vi "Startup.vi"(6 "LabVIEW Web Service":refnum<class "Web Service.lvclass">) -> ()   [LabVIEW 2015]
uses:
  <vilib>/wsapi/Web Service.lvclass
  Configuration/Global_Configurations.vi
panel:
  # "Use the web service input terminal to call the VIs on the Service subpalette of the Web Services palette. Do not remove it from the connector pane unless you don't need access to the palette."
  # "Any additional terminals added to the connector pane of a startup VI will be ignored."
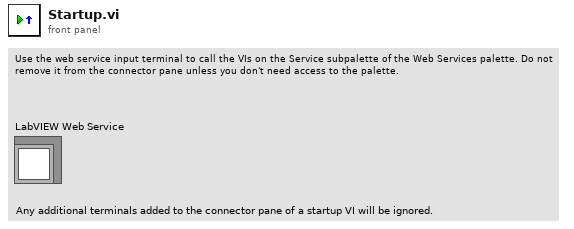
[diagram p1: front panel]
types:
  T1 = cluster{"Path":path, "Name":string, "Authors":string, "Keywords":string, "Description":string, "Cameras":cluster{"Base URL":string, "Path":string, "Name":string}[], "Sampling":cluster{"Sampled Variable":string, "Delta":dbl, "Sampling Freq":u32}[]}[]
  T2 = cluster{"Path":path, "Name":string, "Authors":string, "Keywords":string, "Description":string, "Cameras":cluster{"Base URL":string, "Path":string, "Name":string}[], "Sampling":cluster{"Sampled Variable":string, "Delta":dbl, "Sampling Freq":u32}[]}
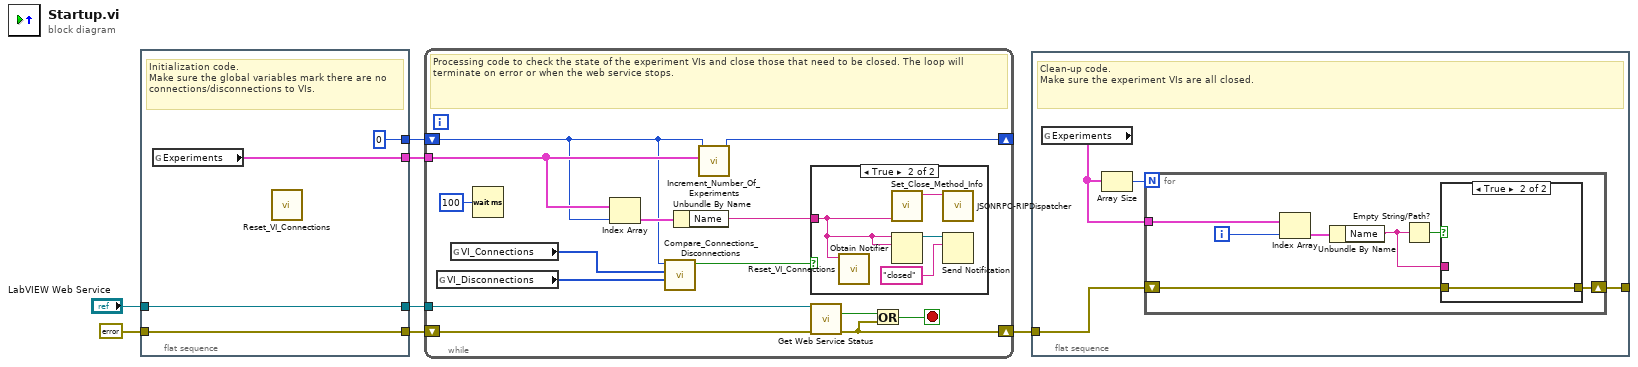
[diagram p0: block diagram]
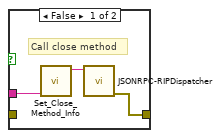
[diagram p2: hidden frame]
diagram:
  n1 = flat-sequence {
    tunnel: "LabVIEW Web Service" -> [w11]
    tunnel: [w11] -> w6
    tunnel: [w10] -> w5
    tunnel: errorcluster {"status"=FALSE, "code"=0, "source"=""} ("error constant") -> [w10]
    tunnel: [0] -> w2
    tunnel: [w8] -> w1
    frame #0 {
      # "Initialization code.\nMake sure the global variables mark there are no connections/disconnections to VIs."
      n2 = global read "Global_Configurations.vi" "Experiments"() -> (w8:T1)
      n3 = call "Reset_VI_Connections.vi"() -> ()  [unwired: 12 in]
    }
  }
  n4 = while {
    tunnel: w6 -> [w24]
    shift-right: [w21] -> w3
    shift-left: w5 -> [w22]
    shift-right: [w18] -> _
    shift-left: w2 -> [w12]
    tunnel: w1 -> [w13]
    stop <- w23 stop-if-true
    # "Processing code to check the state of the experiment VIs and close those that need to be closed. The loop will terminate on error or when the web service stops."
    n5 = global read "Global_Configurations.vi" "VI_Disconnections"() -> (w15:u8[])
    n6 = global read "Global_Configurations.vi" "VI_Connections"() -> (w16:u8[])
    n7 = Wait (ms)(milliseconds to wait=u32 100) -> ()  [unwired: 1 out]
    n8 = Index Array(array=w13, index=w12) -> (element=w19:T2)
    n9 = call "Compare_Connections_Disconnections.vi"("VI_Disconnections"=w15, "VI_Connections"=w16, "Numeric"=w12) -> ("Boolean"=w14:bool)  [unwired: 8 in]
    n10 = Unbundle By Name(w19) -> ("Name"=w17:string)
    n11 = call "Increment_Number_Of_Experiments.vi"("Experiments"=w13, "Numeric"=w12) -> ("f"=w18:i32)  [unwired: 9 in]
    n12 = case shown="True" w14 {
      tunnel: w17 -> [_ w26]
      frame False {
      }
      frame True {
        n13 = call "Reset_VI_Connections.vi"("expId"=w26) -> ()  [unwired: 11 in]
        n14 = call "Set_Close_Method_Info.vi"("expId"=w26) -> ("String"=w29:string)  [unwired: 10 in]
        n15 = Obtain Notifier(name (unnamed)=w26, notification data type=w26) -> (notifier out=w28:refnum<notifier>)  [unwired: 2 in, 2 out]
        n16 = call "JSONRPC-RIPDispatcher.vi"("input string"=w29) -> ()  [unwired: 9 in, 2 out]
        n17 = Send Notification(notification="closed", notifier=w28) -> ()  [unwired: 1 in, 2 out]
      }
    }
    n18 = call <vilib>:"Get Web Service Status.vi"("LabVIEW Web Service"=w24, "error in (no error)"=w22) -> ("service stopping?"=w25:bool, "error out"=w21:errorcluster)  [unwired: 11 in, 1 out]
    n19 = Or(x=w25, y=w21) -> (x .or. y?=w23:bool)
  }
  n20 = flat-sequence {
    tunnel: w3 -> [w32]
    tunnel: [w31] -> _
    frame #0 {
      # "Clean-up code.\nMake sure the experiment VIs are all closed."
      n21 = global read "Global_Configurations.vi" "Experiments"() -> (w30:T1)
      n22 = Array Size(array=w30) -> (size(s)=w33:i32)
      n23 = for {
        N: w33 -> [_]
        shift-right: [w36] -> w31
        shift-left: w32 -> [w35]
        tunnel: w30 -> [w34]
        i -> [w39]
        n24 = Index Array(array=w34, index=w39) -> (element=w40:T2)
        n25 = Unbundle By Name(w40) -> ("Name"=w37:string)
        n26 = Empty String/Path?(string/path=w37) -> (empty?=w38:bool)
        n27 = case shown="True" w38 {
          tunnel: w37 -> [w42 _]
          tunnel: [w41 w44] -> w36
          tunnel: w35 -> [_ w44]
          frame False {
            # "Call close method"
            n28 = call "Set_Close_Method_Info.vi"("expId"=w42) -> ("String"=w43:string)  [unwired: 10 in]
            n29 = call "JSONRPC-RIPDispatcher.vi"("input string"=w43) -> ("error out"=w41:errorcluster)  [unwired: 9 in, 1 out]
          }
          frame True {
          }
        }
      }
    }
  }
